vi "DVR Get VIs.vi"(8 "error in (no error)":errorcluster) -> (0 "error out":errorcluster, 3 "VIs":path[](array[path]))   [LabVIEW 2019, in "Language Selection.lvlib"]
doc: "Converts the Data Value Reference back into Controls translation.\n- - -\nCopyright (c) 2026, Merecs Engineering GmbH"
uses:
  Language Selection.lvlib
  Global Language Selection.vi
panel:
  # "Connector Pane"
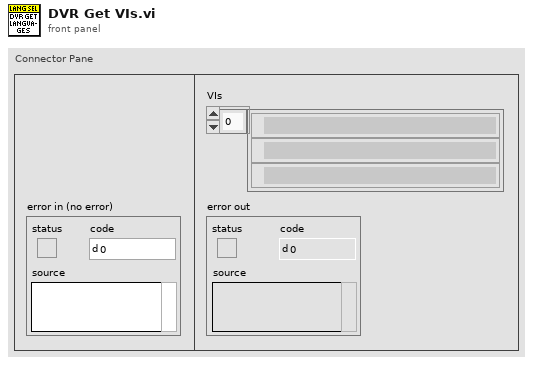
[diagram p1: front panel]
types:
  T1 = typedef "Language Selection.lvlib/Cluster DVR.ctl" = cluster{"Data":T2, "VIs":path[], "FP Translation":map{string, T3}, "Text Translation":map{string, T3}, "Front panels":set{refnum<vi>}}
  T2 = typedef "Language Selection.lvlib/Cluster Settings Data.ctl" = cluster{"Startup Language":string, "Default Language":string, "Languages":cluster{"ANSI":string[], "Unicode":string[]}}
  T3 = typedef "Language Selection.lvlib/Cluster LanguageClusterWithRefnum.ctl" = cluster{"Property":T4[], "Controls":set{refnum<vi>}}
  T4 = typedef "Language Selection.lvlib/Cluster PropertyTranslation.ctl" = cluster{"Type":T5, "Translation ANSI":string[], "Translation Unicode":string[]}
  T5 = typedef "Language Selection.lvlib/Enum Property Type.ctl" = enum16{"NA", "Caption", "String Value", "Boolean Text", "Ring Strings", "1D Array Elements", "2D Array Elements", "(MC)Listbox Header", "(MC)Listbox Items", "Tab Pages Names", "X & Y GraphChart", "Plot Names", "Table Headers", "Table Items", "TipStrip", "Combobox Strings", "Cursor Name", "Tree Col Headers"}
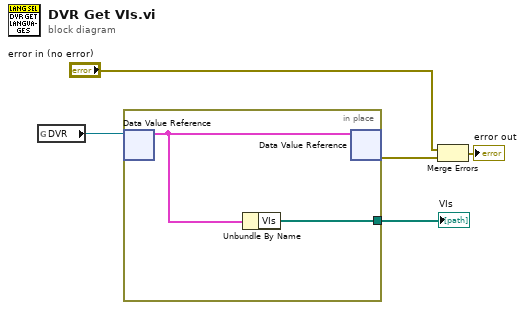
[diagram p0: block diagram]
diagram:
  n1 = global read "Global Language Selection.vi" "DVR"() -> (w2:refnum<data-value>)
  n2 = in-place "In Place Element Structure" {
    in-place-border: [w6] -> w1
    n3 = in-place-dvr #1(w2) -> (w7:T1)  [unwired: 1 out]
    n4 = Unbundle By Name(w7) -> ("VIs"=w6:path[])
    n5 = in-place-dvr #1(w7) -> (w4:errorcluster)  [unwired: 1 out]
  }
  "VIs" <- w1
  n6 = Merge Errors("error in (no error)", w4) -> (→"error out":errorcluster)
